vi "create channels for tags.vi"(7 "outputs?":bool[](array[boolean]), 10 "tags in":T1[](array[typedef]), 11 "EIP Tags Configuration in":refnum<class "EIP Tags Configuration.lvclass">) -> (0 "error out":errorcluster, 2 "channels":refnum<class "EIP Tags Channel.lvclass">[](array[class]), 3 "EIP Tags Configuration out":refnum<class "EIP Tags Configuration.lvclass">)   [LabVIEW 2013, in "EIP Tags editor node.lvclass"]
uses:
  EIP Tags editor node.lvclass
  channel/EIP Tags Channel.lvclass
  configuration/eip tag definition.ctl
  configuration/eip tag types.ctl
  configuration/EIP Tags Configuration.lvclass
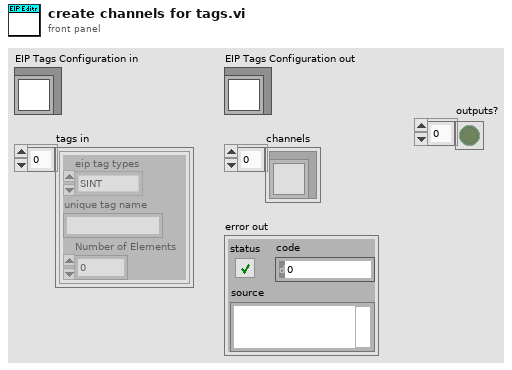
[diagram p1: front panel]
types:
  T1 = typedef "EIP Tags Configuration.lvclass/eip tag definition.ctl" = cluster{"eip tag types":T2, "unique tag name":string, "Number of Elements":u32}
  T2 = typedef "EIP Tags Configuration.lvclass/eip tag types.ctl" = enum16{"SINT", "INT", "DINT", "REAL", "BOOL", "STRING"}
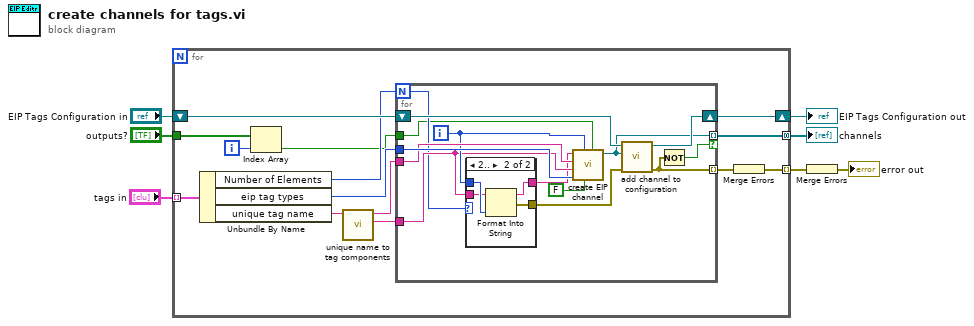
[diagram p0: block diagram]
diagram:
  n1 = for {
    shift-right: [w21] -> w5
    shift-left: "EIP Tags Configuration in" -> [w20]
    tunnel: [w19] -> w7 mode=concatenating
    tunnel: [w16] -> w3 mode=indexing
    tunnel: "tags in" -> [w17] mode=indexing
    tunnel: "outputs?" -> [w10]
    i -> [w8]
    n2 = Unbundle By Name(w17) -> ("Number of Elements"=w15:u32, "eip tag types"=w13:T2, "unique tag name"=w14:string)
    n3 = Index Array(array=w10, index=w8) -> (element=w9:bool)
    n4 = call "unique name to tag components.vi"("unique name"=w14) -> ("Tag Name"=w11:string, "Network Path"=w12:string)  [unwired: 9 in]
    n5 = for {
      N: w15 -> [w24]
      tunnel: [w33] -> w19 mode=indexing if=w31
      tunnel: [w32] -> w18 mode=indexing
      shift-right: [w35] -> w21
      shift-left: w20 -> [w34]
      tunnel: w13 -> [w30]
      tunnel: w12 -> [w29]
      tunnel: w11 -> [w27]
      tunnel: w9 -> [w23]
      i -> [w28]
      n6 = case shown="2.." w24 {
        tunnel: w28 -> [_ w40]
        tunnel: w27 -> [w36 w39]
        tunnel: [w36 w38] -> w26
        tunnel: [_ w37] -> w25
        frame ..1 {
        }
        frame 2.. {
          n7 = Format Into String(initial string=w39, w40) -> (resulting string=w38:string, error out=w37:errorcluster)  [unwired: 2 in]
        }
      }
      n8 = call "create EIP channel.vi"("output?"=w23, "array?"=FALSE, "element index"=w28, "eip tag type"=w30, "Tag Name"=w27, "Network Path"=w29, "name"=w26) -> ("EthernetIP Channel out"=w33:refnum<class "EIP Tags Channel.lvclass">)  [unwired: 4 in]
      n9 = call "add channel to configuration.vi"("error in"=w25, "TBM channel in"=w33, "EthernetIP configuration in"=w34) -> ("error out"=w32:errorcluster, "EthernetIP configuration out"=w35:refnum<class "EIP Tags Configuration.lvclass">)  [unwired: 7 in]
      n10 = Not(x=w32) -> (.not. x?=w31:bool)
    }
    n11 = Merge Errors(w18) -> (w16:errorcluster)
  }
  "channels" <- w7
  "EIP Tags Configuration out" <- w5
  n12 = Merge Errors(w3) -> (→"error out":errorcluster)
